vi "Random Integer.vi"(10 "high":i32, 11 "low":i32) -> (3 "number":i32)   [LabVIEW 2020, in "Full Featured MCP Server.lvlib"]
doc: "Returns a random whole number from low to high, both included. Every number is equally likely."
uses:
  Full Featured MCP Server.lvlib
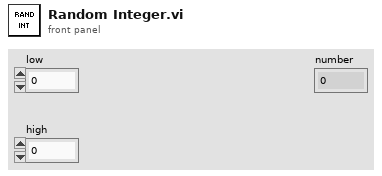
[diagram p1: front panel]
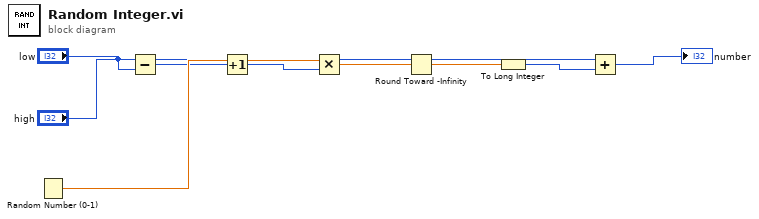
[diagram p0: block diagram]
diagram:
  n1 = Random Number (0-1)() -> (number: 0 to 1=w5:dbl)
  n2 = Subtract(x="high", y="low") -> (x-y=w3:i32)
  n3 = Increment(x=w3) -> (x+1=w4:i32)
  n4 = Multiply(x=w5, y=w4) -> (x*y=w6:dbl)
  n5 = Round Toward -Infinity(1:w6) -> (0:w7:dbl)
  n6 = To Long Integer(number=w7) -> (32bit integer=w8:i32)
  n7 = Add(x="low", y=w8) -> (x+y=→"number":i32)
